vi "ModifyOrder.generated.vi"(11 "buffer.in":u64[](array[numeric])=[0, 0, 0, 0, 0, 0, 0, 0, 0]) -> (3 "OrderBook.Command":T1)   [LabVIEW 2020]
doc: "Cboe PITCH Modify Order (0x27 long, 0x28 short) -> orderbook.command: type ModifyOrder, orderId, new quantity, new price (short price x100 so all prices have 4 implied decimals), nanoseconds, Edit."
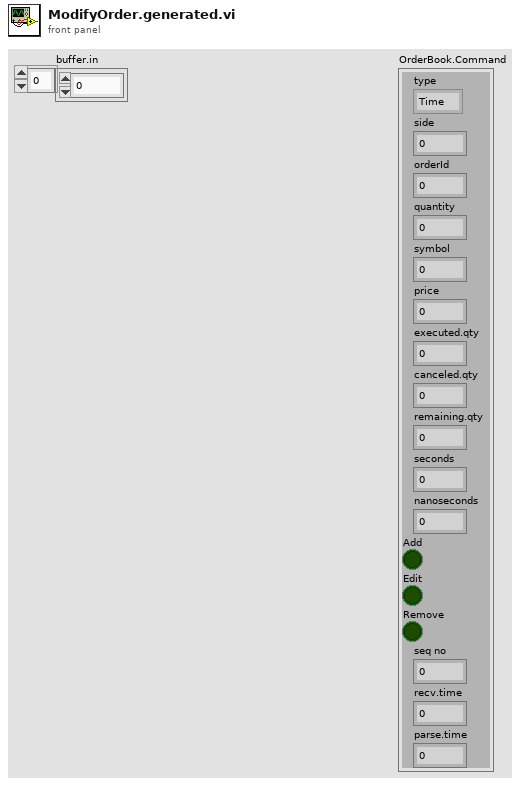
[diagram p1: front panel]
types:
  T1 = cluster{"type":enum8{"Time", "AddOrder", "OrderExecuted", "OrderExecutedAtPrice", "ReduceSize", "ModifyOrder", "DeleteOrder", "Get.Everything", "Get.All.Orders", "Get.Top", "Trade", "Unsupported"}, "side":u8, "orderId ":u64, "quantity":u32, "symbol":u64, "price":u64, "executed.qty":u32, "canceled.qty":u32, "remaining.qty":u32, "seconds":u64, "nanoseconds":u64, "Add":bool, "Edit":bool, "Remove":bool, "seq no":u32, "recv.time":u64, "parse.time":u64}
  T2 = enum8{"Time", "AddOrder", "OrderExecuted", "OrderExecutedAtPrice", "ReduceSize", "ModifyOrder", "DeleteOrder", "Get.Everything", "Get.All.Orders", "Get.Top", "Trade", "Unsupported"}
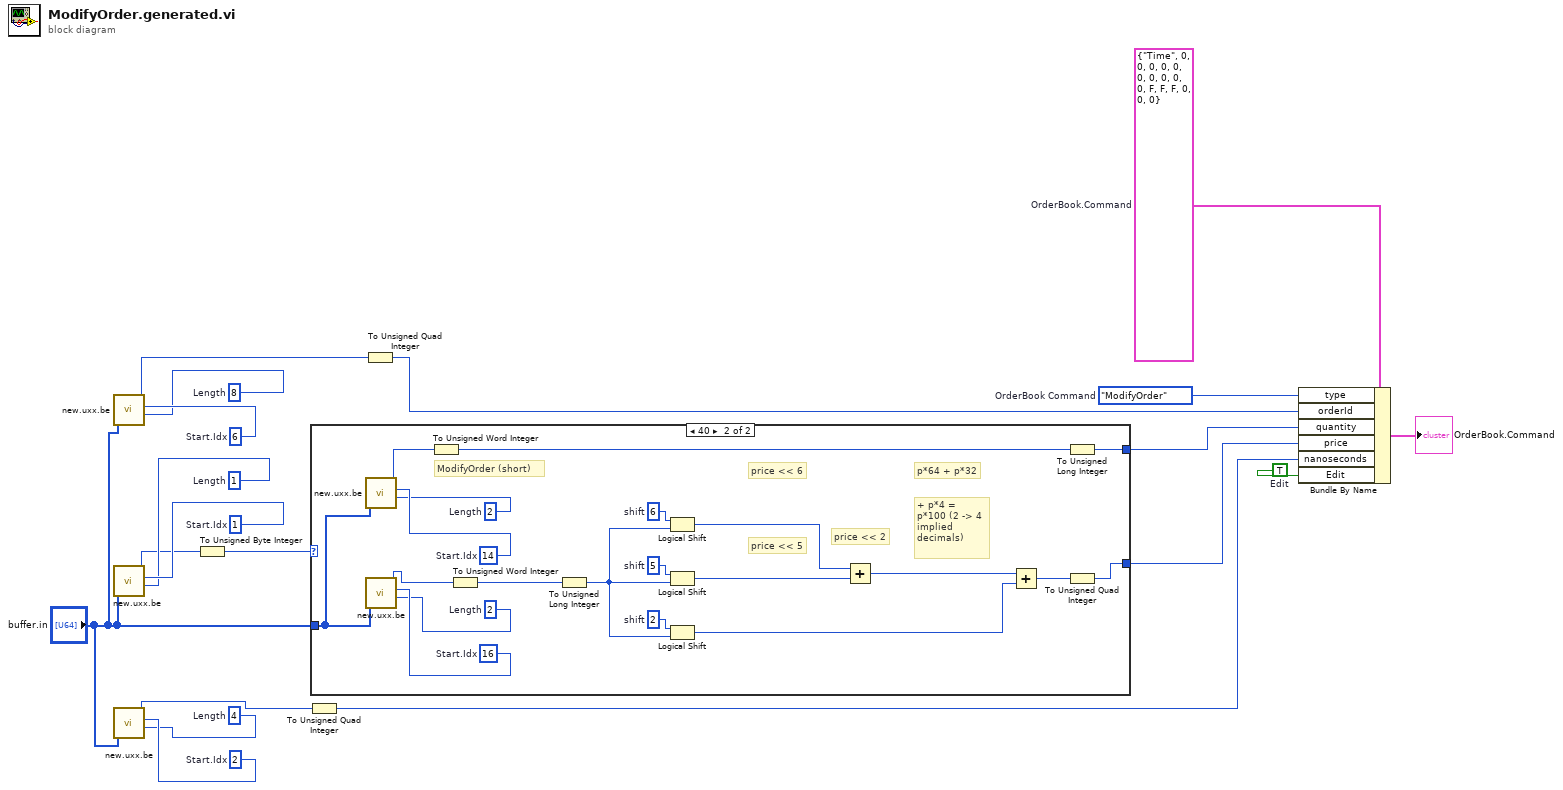
[diagram p0: block diagram]
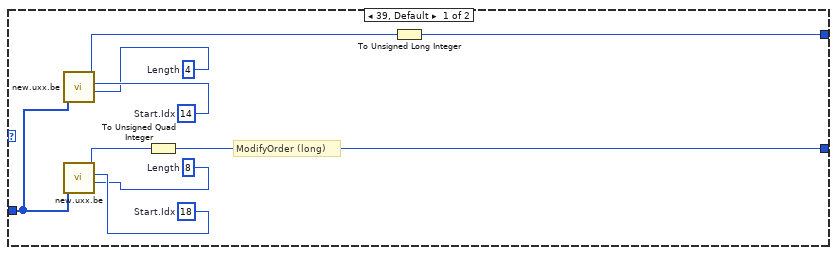
[diagram p2: hidden frame]
diagram:
  w12 = u8 8  # Length
  w13 = u8 6  # Start.Idx
  w15 = u8 4  # Length
  w16 = u8 2  # Start.Idx
  w18 = u8 1  # Length
  w19 = u8 1  # Start.Idx
  w3 = TRUE  # Edit
  w8 = T2."ModifyOrder"  # OrderBook Command
  w2 = T1 {"type"=enum."Time", "side"=0, "orderId "=0, "quantity"=0, "symbol"=0, "price"=0, "executed.qty"=0, "canceled.qty"=0, "remaining.qty"=0, "seconds"=0, "nanoseconds"=0, "Add"=FALSE, "Edit"=FALSE, "Remove"=FALSE, "seq no"=0, "recv.time"=0, "parse.time"=0}  # OrderBook.Command
  n1 = call "new.uxx.be.vi"("buffer (U64)"="buffer.in", "Start.Idx"=w13, "Length"=w12) -> ("Out.Value U64"=w11:u64)  [unwired: 7 in]
  n2 = call "new.uxx.be.vi"("buffer (U64)"="buffer.in", "Start.Idx"=w19, "Length"=w18) -> ("Out.Value U64"=w17:u64)  [unwired: 7 in]
  n3 = call "new.uxx.be.vi"("buffer (U64)"="buffer.in", "Start.Idx"=w16, "Length"=w15) -> ("Out.Value U64"=w14:u64)  [unwired: 7 in]
  n4 = To Unsigned Byte Integer(number=w17) -> (unsigned 8bit integer=w9:u8)
  n5 = To Unsigned Quad Integer(1:w14) -> (0:w4:u64)
  n6 = case shown="40" w9 {
    tunnel: "buffer.in" -> [w25 w44]
    tunnel: [w21 w30] -> w6
    tunnel: [w20 w29] -> w5
    frame 39, Default {
      w23 = u8 8  # Length
      w24 = u8 18  # Start.Idx
      w27 = u8 4  # Length
      w28 = u8 14  # Start.Idx
      # "ModifyOrder (long)"
      n7 = call "new.uxx.be.vi"("buffer (U64)"=w25, "Start.Idx"=w28, "Length"=w27) -> ("Out.Value U64"=w26:u64)  [unwired: 7 in]
      n8 = call "new.uxx.be.vi"("buffer (U64)"=w25, "Start.Idx"=w24, "Length"=w23) -> ("Out.Value U64"=w22:u64)  [unwired: 7 in]
      n9 = To Unsigned Quad Integer(1:w22) -> (0:w20:u64)
      n10 = To Unsigned Long Integer(number=w26) -> (unsigned 32bit integer=w21:u32)
    }
    frame 40 {
      w37 = i16 2  # shift
      w38 = i16 5  # shift
      w39 = i16 6  # shift
      w42 = u8 2  # Length
      w43 = u8 16  # Start.Idx
      w47 = u8 2  # Length
      w48 = u8 14  # Start.Idx
      # "+ p*4 = p*100 (2 -> 4 implied decimals)"
      # "p*64 + p*32"
      # "price << 2"
      # "price << 5"
      # "price << 6"
      # "ModifyOrder (short)"
      n11 = call "new.uxx.be.vi"("buffer (U64)"=w44, "Start.Idx"=w48, "Length"=w47) -> ("Out.Value U64"=w46:u64)  [unwired: 7 in]
      n12 = call "new.uxx.be.vi"("buffer (U64)"=w44, "Start.Idx"=w43, "Length"=w42) -> ("Out.Value U64"=w41:u64)  [unwired: 7 in]
      n13 = To Unsigned Word Integer(number=w46) -> (unsigned 16bit integer=w45:u16)
      n14 = To Unsigned Word Integer(number=w41) -> (unsigned 16bit integer=w40:u16)
      n15 = To Unsigned Long Integer(number=w40) -> (unsigned 32bit integer=w36:u32)
      n16 = Logical Shift(y=w39, x=w36) -> (x << y=w35:u32)
      n17 = Logical Shift(y=w38, x=w36) -> (x << y=w34:u32)
      n18 = Logical Shift(y=w37, x=w36) -> (x << y=w32:u32)
      n19 = Add(x=w35, y=w34) -> (x+y=w33:u32)
      n20 = Add(x=w33, y=w32) -> (x+y=w31:u32)
      n21 = To Unsigned Long Integer(number=w45) -> (unsigned 32bit integer=w30:u32)
      n22 = To Unsigned Quad Integer(1:w31) -> (0:w29:u64)
    }
  }
  n23 = To Unsigned Quad Integer(1:w11) -> (0:w7:u64)
  n24 = Bundle By Name(cluster=w2, "type"=w8, "orderId"=w7, "quantity"=w6, "price"=w5, "nanoseconds"=w4, "Edit"=w3) -> (→"OrderBook.Command":T1)
